vi "Write_Raw.vi"(7 "n frames":u32, 8 "error in (no error)":errorcluster, 9 "length":i32, 10 "bytes in":u8[](array[numeric]), 11 "channel in":refnum<class "CANsub_Channel.lvclass">) -> (0 "error out":errorcluster, 2 "bytes out":u8[](array[numeric]), 3 "channel out":refnum<class "CANsub_Channel.lvclass">)   [LabVIEW 2021, in "CANsub_API.lvlib" / "CANsub_Channel.lvclass"]
doc: "Sends a buffer of WebSocket frames that the caller prepared (for example with C_CIF_Encode_RT) with one TCP Write. length is the number of valid bytes in bytes in. n frames is the number of CAN frames in the buffer; it is added to frames written in the status. Loop-safe: no allocation in this class, bounded time (TCP Write timeout 1 s)."
uses:
  CANsub_Channel.lvclass
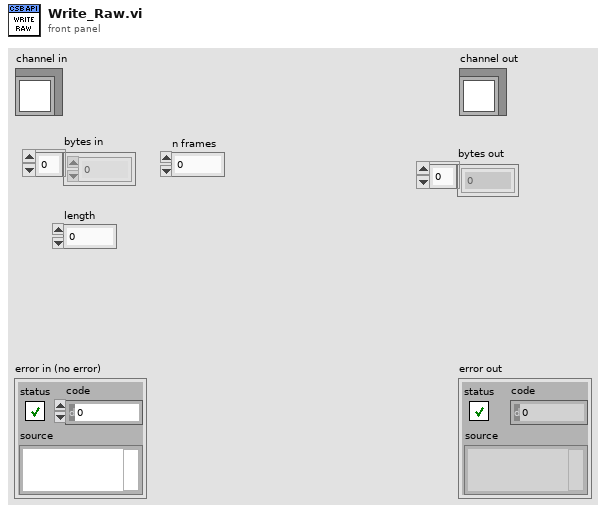
[diagram p1: front panel]
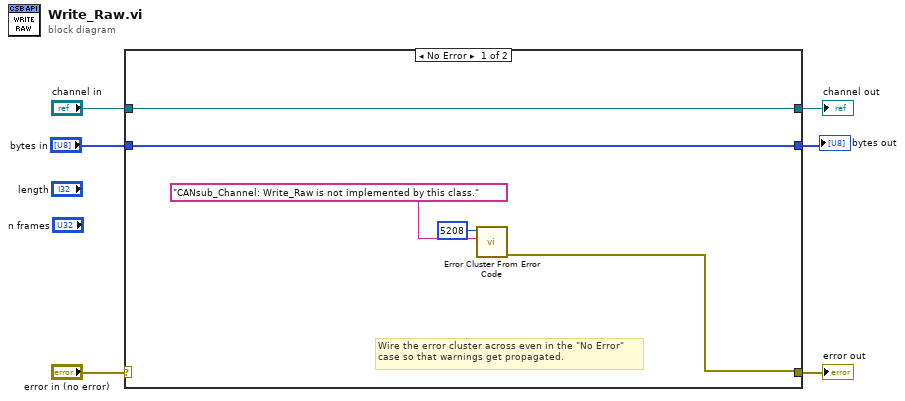
[diagram p0: block diagram]
diagram:
  n1 = case shown="No Error" "error in (no error)" {
    selector: "error in (no error)" -> [_ w14]
    tunnel: [w7 w14] -> w5
    tunnel: [w11 w13] -> w3
    tunnel: "channel in" -> [w11 w13]
    tunnel: [w10 w12] -> w2
    tunnel: "bytes in" -> [w10 w12]
    frame No Error {
      # "Wire the error cluster across even in the \"No Error\"\ncase so that warnings get propagated."
      n2 = call <vilib>:"Error Cluster From Error Code.vi"("error message (\"\")"="CANsub_Channel: Write_Raw is not implemented by this class." ("error message (\"\")"), "error code (0)"=5208) -> ("error out"=w7:errorcluster)  [unwired: 7 in]
    }
    frame Error {
    }
  }
  "error out" <- w5
  "channel out" <- w3
  "bytes out" <- w2
